vi "RDC-Probe-Calculate_Dimensions.vi"(9 "Dieletrisk konstant":dbl=2.53, 10 "Core Diameter [mm]":dbl=3.5) -> (1 "50ohm Probe Impedane?":bool, 2 "probe Impedanse":dbl, 3 "Probe Parameters 2":T1={"lenght [mm]"=50.0, "Core Diameter [mm]"=0.93, "Inner Diameter [mm]"=3.5, "Dieletrisk constant"=2.53})   [LabVIEW 2020, in "RDC-Reflection_Data_Computation.lvlib"]
doc: "Computes the probe parameters cluster and the probe impedance from a core diameter in mm and a dielectric constant. Reports whether the impedance is 50 ohm."
uses:
  RDC-Reflection_Data_Computation.lvlib
  RDC-Probe_parameters.ctl
panel:
  out "Inner Diameter [mm]":dbl=0.93
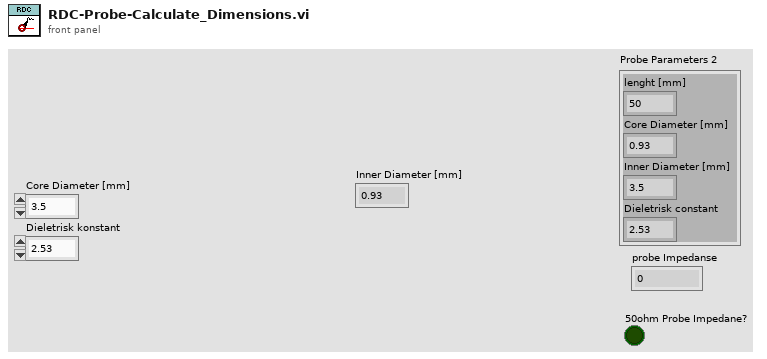
[diagram p1: front panel]
types:
  T1 = typedef "RDC-Reflection_Data_Computation.lvlib/RDC-Probe_parameters.ctl" = cluster{"lenght [mm]":dbl, "Core Diameter [mm]":dbl, "Inner Diameter [mm]":dbl, "Dieletrisk constant":dbl}
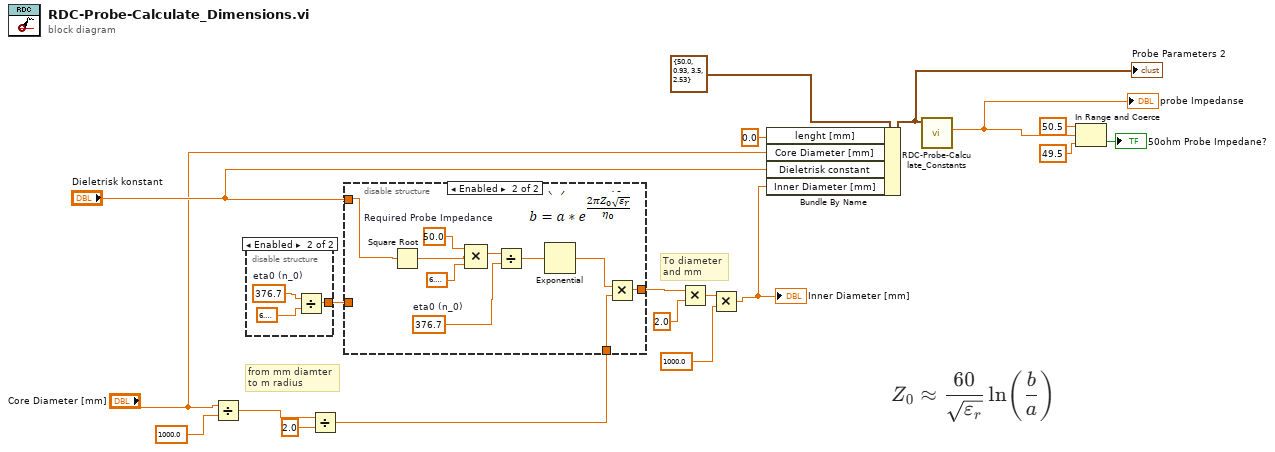
[diagram p0: block diagram]
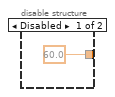
[diagram p2: hidden frame]
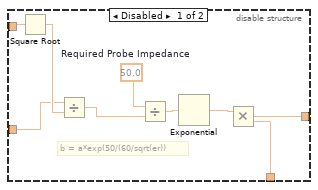
[diagram p3: hidden frame]
diagram:
  # "from mm diamter \nto m radius"
  # "To diameter \nand mm"
  n1 = Divide(x="Core Diameter [mm]", y=1000.0) -> (x/y=w18:dbl)
  n2 = disable-structure shown="Enabled" {
    disable-tunnel: [60.0 ("x") w21] -> w1
    frame Disabled {
    }
    frame Enabled {
      w22 = 376.7  # eta0 (n_0)
      n3 = Divide(x=w22, y=6.283185307179586) -> (x/y=w21:dbl)
    }
  }
  n4 = Divide(x=w18, y=2.0) -> (x/y=w16:dbl)
  n5 = disable-structure shown="Enabled" {
    disable-tunnel: w16 -> [w27 w41]
    disable-tunnel: [w26 w40] -> w15
    disable-tunnel: "Dieletrisk konstant" -> [w25 w42]
    disable-tunnel: w1 -> [w24 _]
    frame Disabled {
      w30 = 50.0  # Required Probe Impedance
      # "b = a*exp(50/(60/sqrt(er))"
      n6 = Square Root(x=w25) -> (sqrt(x)=w32:dbl)
      n7 = Divide(x=w24, y=w32) -> (x/y=w31:dbl)
      n8 = Divide(x=w30, y=w31) -> (x/y=w29:dbl)
      n9 = Exponential(1:w29) -> (0:w28:dbl)
      n10 = Multiply(x=w28, y=w27) -> (x*y=w26:dbl)
    }
    frame Enabled {
      w34 = 376.7  # eta0 (n_0)
      w37 = 50.0  # Required Probe Impedance
      n11 = Square Root(x=w42) -> (sqrt(x)=w36:dbl)
      n12 = Compound Arithmetic op=MULTIPLY(w37, w36, 6.283185307179586) -> (w35:dbl)
      n13 = Divide(x=w35, y=w34) -> (x/y=w39:dbl)
      n14 = Exponential(1:w39) -> (0:w38:dbl)
      n15 = Multiply(x=w38, y=w41) -> (x*y=w40:dbl)
    }
  }
  n16 = Multiply(x=w15, y=2.0) -> (x*y=w13:dbl)
  n17 = Multiply(x=w13, y=1000.0) -> (x*y=w7:dbl)
  "Inner Diameter [mm]" <- w7
  n18 = Bundle By Name(cluster=T1 {"lenght [mm]"=50.0, "Core Diameter [mm]"=0.93, "Inner Diameter [mm]"=3.5, "Dieletrisk constant"=2.53} ("Probe Parameters"), "lenght [mm]"=0.0, "Core Diameter [mm]"="Core Diameter [mm]", "Dieletrisk constant"="Dieletrisk konstant", "Inner Diameter [mm]"=w7) -> (w2:T1)
  "Probe Parameters 2" <- w2
  n19 = call "RDC-Probe-Calculate_Constants.vi"("Probe Parameters"=w2) -> ("probe Impedanse"=w6:dbl)  [unwired: 8 in, 2 out]
  "probe Impedanse" <- w6
  n20 = In Range and Coerce(upper limit=50.5, x=w6, lower limit=49.5 ("upper limit")) -> (In Range?=→"50ohm Probe Impedane?":bool)  [unwired: 1 out]
